vi "SMR_LabVIEW_V3.vi"() -> ()   [LabVIEW 2025]
uses:
  <vilib>/DAQmx/read.llb/DAQmx Read (Analog 1D DBL NChan 1Samp).vi
  <vilib>/DAQmx/create/channels.llb/DAQmx Create Channel (AI-Temperature-Thermocouple).vi
  <vilib>/DAQmx/create/channels.llb/DAQmx Create Channel (AI-Voltage-Basic).vi
  <vilib>/DAQmx/miscellaneous.llb/DAQmx Fill In Error Info.vi
panel:
  in  "Flow CSV Path":path
  in  "Pressure CSV Path":path
  in  "Temeprature CSV Path":path
  out "Heat Exchanger Pressure History":dbl(graph)
  out "Main Loop Pressure History":T1(graph)
  out "Heat Exchanger Temperature History":cluster{"Waveform":dbl, "Waveform":dbl}(graph)
  out "Main Loop Temeperature History":T2(graph)
  out "Overall Avg Pressure (psi)":dbl
  out "Heat Exchanger Pressure P6 (psi)":dbl
  out "Main Loop Avg Pressure (psi)":dbl
  out "Heat Exchanger Avg Temp (deg C)":dbl
  out "Main Loop Avg Temp (deg C)":dbl
  out "Raw NI9201 \nVoltage Display":T3
  out "Temperature Display":T4
  out "Pressure Display":T5
  in  "Flow Offset Correction (GPM)":dbl=-0.3
  out "Flow History":dbl(graph)
  out "Overall Pressure History":T6(graph)
  out "Overall Temperature History":T7(graph)
  out "Max Loop Pressure (psi)":dbl
  out "Overall Avg Temp (deg C)":dbl
  out "Max Loop Temp (deg C)":dbl
  out "Heat Exchanger Flow (GPM)":dbl
  in  "Loop Period (ms)":dbl=1000.0
  in  "Stop":bool
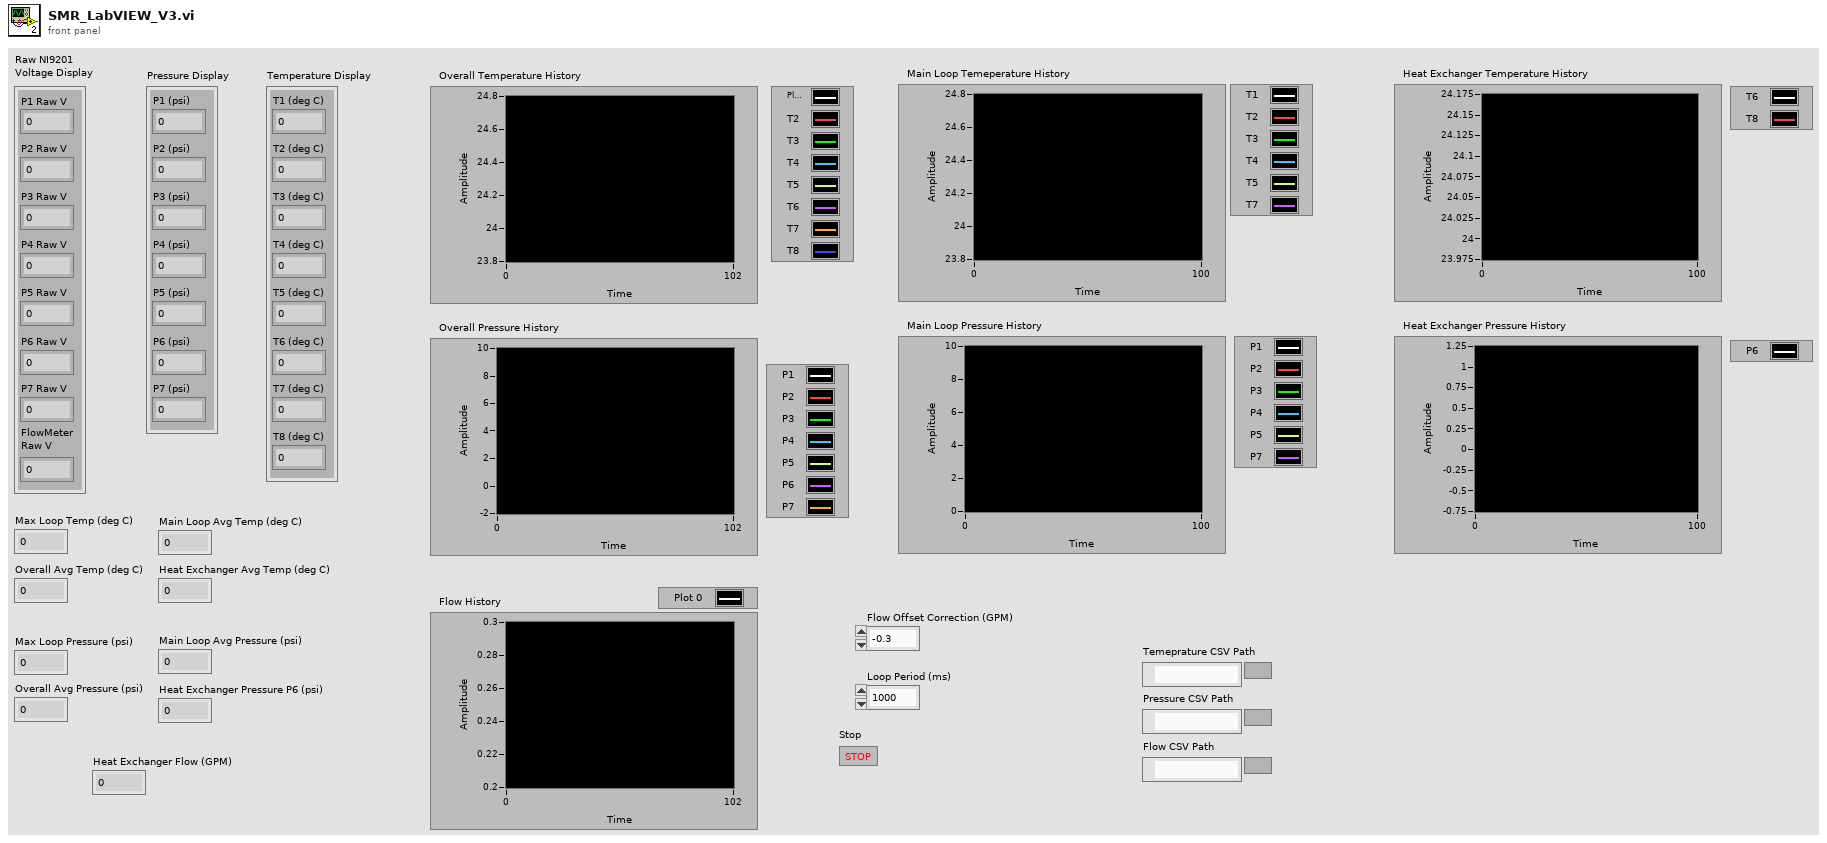
[diagram p1: front panel]
types:
  T1 = cluster{"P1":dbl, "P2":dbl, "P3":dbl, "P4":dbl, "P5":dbl, "P7":dbl}
  T2 = cluster{"Waveform":dbl, "Waveform":dbl, "Waveform":dbl, "Waveform":dbl, "Waveform":dbl, "Waveform":dbl}
  T3 = cluster{"P1 Raw V":dbl, "P2 Raw V":dbl, "P3 Raw V":dbl, "P4 Raw V":dbl, "P5 Raw V":dbl, "P6 Raw V":dbl, "P7 Raw V":dbl, "FlowMeter\nRaw V":dbl}
  T4 = cluster{"T1 (deg C)":dbl, "T2 (deg C)":dbl, "T3 (deg C)":dbl, "T4 (deg C)":dbl, "T5 (deg C)":dbl, "T6 (deg C)":dbl, "T7 (deg C)":dbl, "T8 (deg C)":dbl}
  T5 = cluster{"P1 (psi)":dbl, "P2 (psi)":dbl, "P3 (psi)":dbl, "P4 (psi)":dbl, "P5 (psi)":dbl, "P6 (psi)":dbl, "P7 (psi)":dbl}
  T6 = cluster{"P1":dbl, "P2":dbl, "P3":dbl, "P4":dbl, "P5":dbl, "P6":dbl, "P7":dbl}
  T7 = cluster{"Waveform":dbl, "Waveform":dbl, "Waveform":dbl, "Waveform":dbl, "Waveform":dbl, "Waveform":dbl, "Waveform":dbl, "Waveform":dbl}
  T8 = enum16{"open", "replace", "create", "open or create", "replace or create", "replace or create with confirmation"}
  T9 = cluster{"P1":dbl, "P2":dbl, "P3":dbl, "P4":dbl, "P5":dbl, "P6":dbl, "P7":dbl, "Flow":dbl}
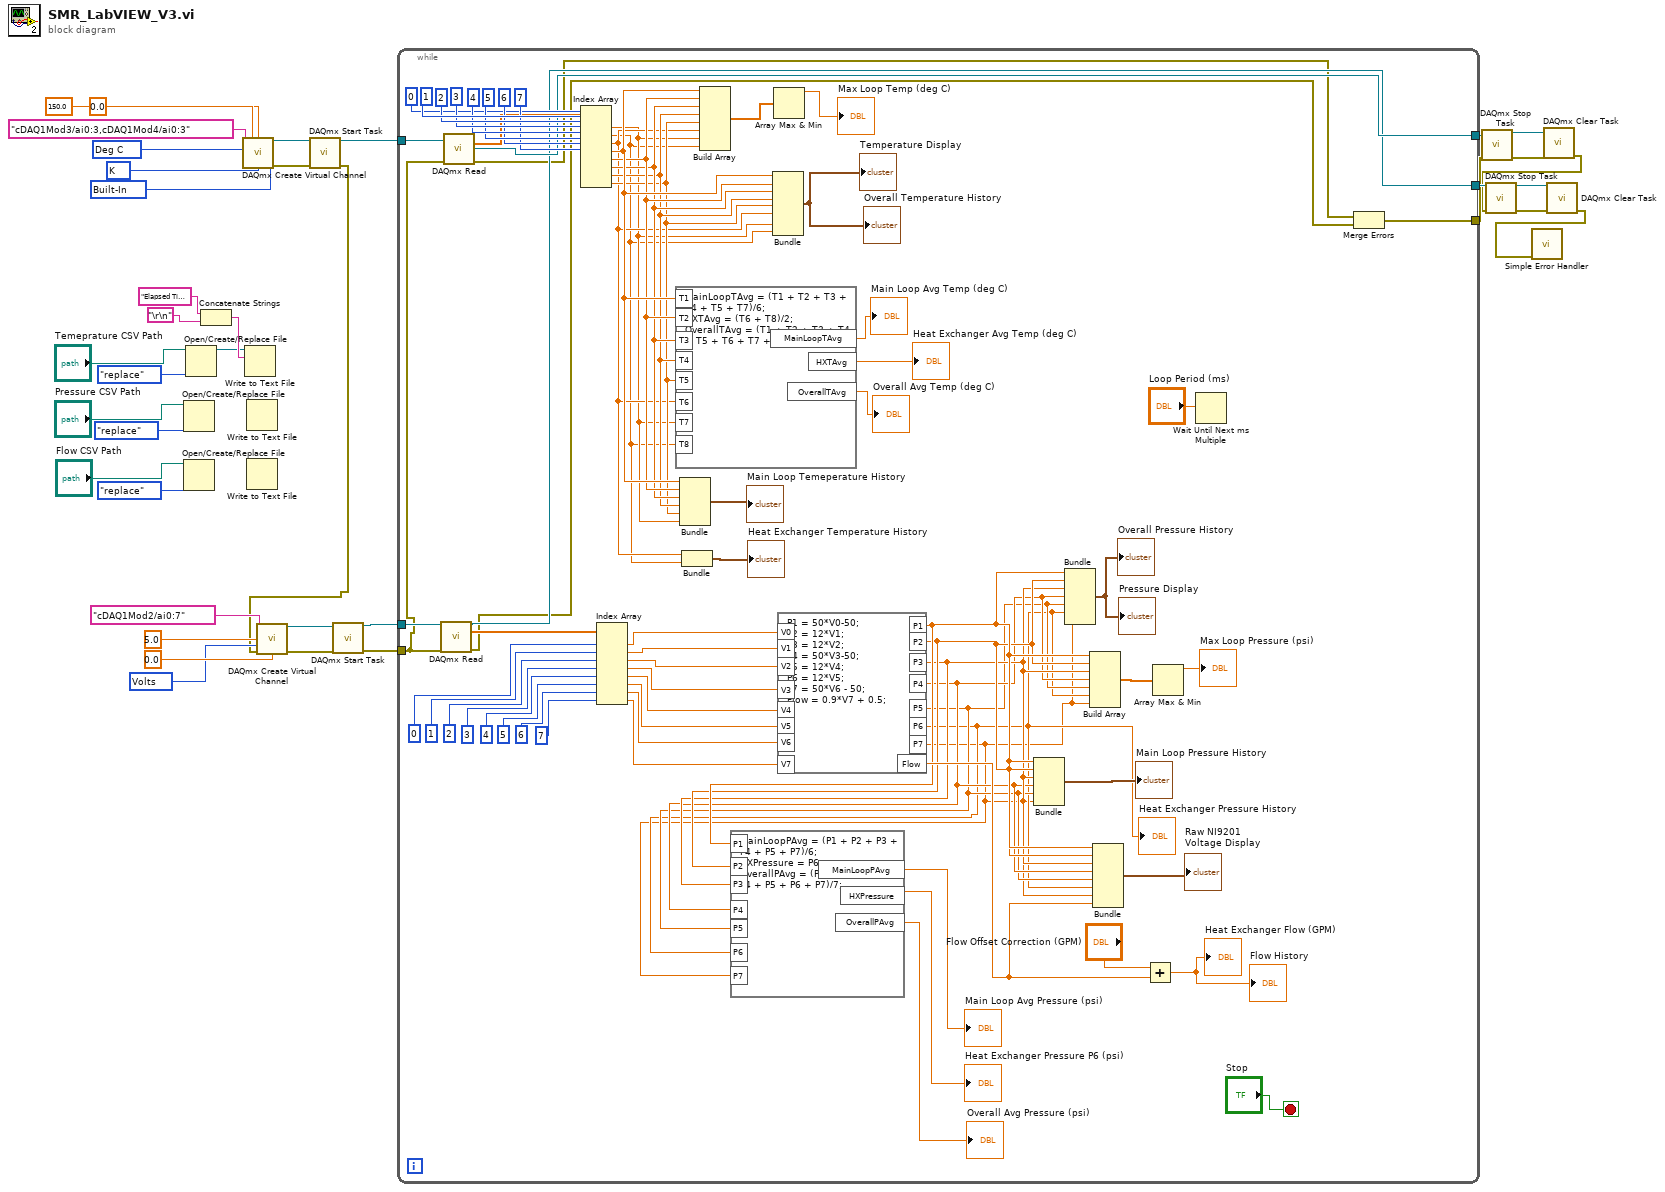
[diagram p0: block diagram]
diagram:
  w25 = 10200 items=["Built-In"=10200, "Constant Value"=10116, "Channel"=10113] ("cjc source")
  w26 = 10073 items=["J"=10072, "K"=10073, "N"=10077, "R"=10082, "S"=10085, "T"=10086, "B"=10047, "E"=10055] ("thermocouple type")
  w27 = 10143 items=["Deg C"=10143, "Deg F"=10144, "Kelvins"=10325, "Deg R"=10145, "From Custom Scale"=10065] ("units")
  w34 = 10348 items=["Volts"=10348, "From Custom Scale"=10065] ("units")
  n1 = Open/Create/Replace File(file path (use dialog)="Pressure CSV Path", operation (0:open)=T8."replace") -> ()  [unwired: 4 in, 3 out]
  n2 = Open/Create/Replace File(file path (use dialog)="Flow CSV Path", operation (0:open)=T8."replace") -> ()  [unwired: 4 in, 3 out]
  n3 = Open/Create/Replace File(file path (use dialog)="Temeprature CSV Path", operation (0:open)=T8."replace") -> (refnum out=w1:refnum<file>)  [unwired: 4 in, 2 out]
  n4 = Concatenate Strings("Elapsed Time (s),T1 (deg C),T2 (deg C),T3 (deg C),T4 (deg C),T5 (deg C),T6 (deg C),T7 (deg C),T8 (deg C),Main Loop Avg Temp (deg C),HX Avg Temp (deg C),Overall Avg Temp (deg C)", "\r\n") -> (w2:string)
  n5 = call-poly <vilib>:"DAQmx Create Virtual Channel.vi"("maximum value"=150.0, "minimum value"=0.0, "physical channels"=tag "cDAQ1Mod3/ai0:3,cDAQ1Mod4/ai0:3", "cjc source"=w25, "units"=w27, "thermocouple type"=w26) -> ("task out"=w24:refnum<k21>, "error out"=w23:errorcluster)  [unwired: 8 in]
  n6 = Write to Text File(file (use dialog)=w1, text=w2) -> ()  [unwired: 2 in, 3 out]
  n7 = Write to Text File() -> ()  [unwired: 4 in, 3 out]
  n8 = Write to Text File() -> ()  [unwired: 4 in, 3 out]
  n9 = call <vilib>:"DAQmx Start Task.vi"("task/channels in"=w24, "error in"=w23) -> ("task out"=w22:refnum<k21>, "error out"=w18:errorcluster)  [unwired: 12 in]
  n10 = call-poly <vilib>:"DAQmx Create Virtual Channel.vi"("maximum value"=5.0, "minimum value"=0.0, "physical channels"=tag "cDAQ1Mod2/ai0:7", "units"=w34, "error in"=w18) -> ("task out"=w33:refnum<k21>, "error out"=w32:errorcluster)  [unwired: 9 in]
  n11 = call <vilib>:"DAQmx Start Task.vi"("task/channels in"=w33, "error in"=w32) -> ("task out"=w31:refnum<k21>, "error out"=w20:errorcluster)  [unwired: 12 in]
  n12 = while {
    tunnel: w31 -> [w103]
    tunnel: w22 -> [w68]
    tunnel: [w50] -> w21
    tunnel: w20 -> [w41]
    tunnel: [w42] -> w19
    tunnel: [w38] -> w17
    stop <- "Stop" stop-if-true
    n13 = call-poly <vilib>:"DAQmx Read.vi"("task/channels in"=w103, "error in"=w41) -> ("task out"=w42:refnum<k21>, "data"=w94:dbl[], "error out"=w39:errorcluster)  [unwired: 11 in]
    n14 = call-poly <vilib>:"DAQmx Read.vi"("task/channels in"=w68, "error in"=w41) -> ("task out"=w50:refnum<k21>, "data"=w59:dbl[], "error out"=w40:errorcluster)  [unwired: 11 in]
    n15 = Index Array(array=w59, index #1=0 ("index"), index #2=1 ("index"), index #3=2 ("index"), index #4=3 ("index"), index #5=4 ("index"), index #6=5 ("index"), index #7=6 ("index"), index #8=7 ("index")) -> (element #1=w52:dbl, element #2=w51:dbl, element #3=w53:dbl, element #4=w58:dbl, element #5=w57:dbl, element #6=w56:dbl, element #7=w55:dbl, element #8=w54:dbl)
    n16 = Index Array(array=w94, index #1=0 ("index"), index #2=1 ("index"), index #3=2 ("index"), index #4=3 ("index"), index #5=4 ("index"), index #6=5 ("index"), index #7=6 ("index"), index #8=7 ("index")) -> (element #1=w93:dbl, element #2=w92:dbl, element #3=w91:dbl, element #4=w90:dbl, element #5=w89:dbl, element #6=w88:dbl, element #7=w87:dbl, element #8=w86:dbl)
    n17 = formula code="MainLoopTAvg = (T1 + T2 + T3 + T4 + T5 + T7)/6;\nHXTAvg = (T6 + T8)/2;\nOverallTAvg = (T1 + T2 + T3 + T4 + T5 + T6 + T7 + T8)/8;"("T1"=w58, "T2"=w57, "T3"=w56, "T4"=w55, "T5"=w54, "T6"=w53, "T7"=w52, "T8"=w51) -> ("MainLoopTAvg"=→"Main Loop Avg Temp (deg C)":dbl, "HXTAvg"=→"Heat Exchanger Avg Temp (deg C)":dbl, "OverallTAvg"=→"Overall Avg Temp (deg C)":dbl)
    n18 = Bundle("Waveform"=w58, "Waveform"=w57, "Waveform"=w56, "Waveform"=w55, "Waveform"=w54, "Waveform"=w52) -> (→"Main Loop Temeperature History":T2)  [unwired: 1 in]
    n19 = Bundle("Waveform"=w53, "Waveform"=w51) -> (→"Heat Exchanger Temperature History":cluster{"Waveform":dbl, "Waveform":dbl})  [unwired: 1 in]
    n20 = Build Array(w58, w57, w56, w55, w54, w53, w52, w51) -> (w104:dbl[])
    n21 = Bundle("Waveform"=w58, "Waveform"=w57, "Waveform"=w56, "Waveform"=w55, "Waveform"=w54, "Waveform"=w53, "Waveform"=w52, "Waveform"=w51) -> (→"Overall Temperature History" →"Temperature Display":T7)  [unwired: 1 in]
    n22 = Array Max & Min(array=w104) -> (max value=→"Max Loop Temp (deg C)":dbl)  [unwired: 3 out]
    n23 = formula code="P1 = 50*V0-50;\nP2 = 12*V1;\nP3 = 12*V2;\nP4 = 50*V3-50;\nP5 = 12*V4;\nP6 = 12*V5; \nP7 = 50*V6 - 50;\nFlow = 0.9*V7 + 0.5;"("V0"=w93, "V1"=w92, "V2"=w91, "V3"=w90, "V4"=w89, "V5"=w88, "V6"=w87, "V7"=w86) -> ("P1"=w49:dbl, "P2"=w48:dbl, "P3"=w47:dbl, "P4"=w46:dbl, "P5"=w45:dbl, "P6"=w44:dbl, "P7"=w43:dbl, "Flow"=w79:dbl)
    "Heat Exchanger Pressure History" <- w44
    n24 = formula code="MainLoopPAvg = (P1 + P2 + P3 + P4 + P5 + P7)/6;\nHXPressure = P6;\nOverallPAvg = (P1 + P2 + P3 + P4 + P5 + P6 + P7)/7;"("P1"=w49, "P2"=w48, "P3"=w47, "P4"=w46, "P5"=w45, "P6"=w44, "P7"=w43) -> ("MainLoopPAvg"=→"Main Loop Avg Pressure (psi)":dbl, "HXPressure"=→"Heat Exchanger Pressure P6 (psi)":dbl, "OverallPAvg"=→"Overall Avg Pressure (psi)":dbl)
    n25 = Bundle("P1"=w49, "P2"=w48, "P3"=w47, "P4"=w46, "P5"=w45, "P7"=w43) -> (→"Main Loop Pressure History":T1)  [unwired: 1 in]
    n26 = Bundle("P1"=w49, "P2"=w48, "P3"=w47, "P4"=w46, "P5"=w45, "P6"=w44, "P7"=w43) -> (→"Overall Pressure History" →"Pressure Display":T6)  [unwired: 1 in]
    n27 = Build Array(w49, w48, w47, w46, w45, w44, w43) -> (w82:dbl[])
    n28 = Bundle("P1"=w49, "P2"=w48, "P3"=w47, "P4"=w46, "P5"=w45, "P6"=w44, "P7"=w43, "Flow"=w79) -> (→"Raw NI9201 \nVoltage Display":T9)  [unwired: 1 in]
    n29 = Add(x="Flow Offset Correction (GPM)", y=w79) -> (x+y=→"Heat Exchanger Flow (GPM)" →"Flow History":dbl)
    n30 = Array Max & Min(array=w82) -> (max value=→"Max Loop Pressure (psi)":dbl)  [unwired: 3 out]
    n31 = Wait Until Next ms Multiple(millisecond multiple="Loop Period (ms)") -> ()  [unwired: 1 out]
    n32 = Merge Errors(w40, w39) -> (w38:errorcluster)
  }
  n33 = call <vilib>:"DAQmx Stop Task.vi"("task/channels in"=w21, "error in"=w17) -> ("task out"=w16:refnum<k21>, "error out"=w14:errorcluster)  [unwired: 12 in]
  n34 = call <vilib>:"DAQmx Clear Task.vi"("task in"=w16, "error in"=w14) -> ("error out"=w13:errorcluster)  [unwired: 13 in]
  n35 = call <vilib>:"DAQmx Stop Task.vi"("task/channels in"=w19, "error in"=w13) -> ("task out"=w15:refnum<k21>, "error out"=w12:errorcluster)  [unwired: 12 in]
  n36 = call <vilib>:"DAQmx Clear Task.vi"("task in"=w15, "error in"=w12) -> ("error out"=w11:errorcluster)  [unwired: 13 in]
  n37 = call <vilib>:"Simple Error Handler.vi"("error in (no error)"=w11) -> ()  [unwired: 4 in, 5 out]
